vi "Cmd HO (TT).vi"(8 "error in (no error)":errorcluster caption="에러 입력(에러 없음)", 11 "AUDIX EM1000 입력":refnum<class "AUDIX EM1000.lvclass">) -> (0 "error out":errorcluster caption="에러 출력", 3 "AUDIX EM1000 출력":refnum<class "AUDIX EM1000.lvclass">)   [LabVIEW 2023, in "Turn Table and Mast.lvlib" / "AUDIX EM1000.lvclass"]
uses:
  AUDIX EM1000.lvclass
  AUDIX EM1000.lvclass/AUDIX EM1000.ctl
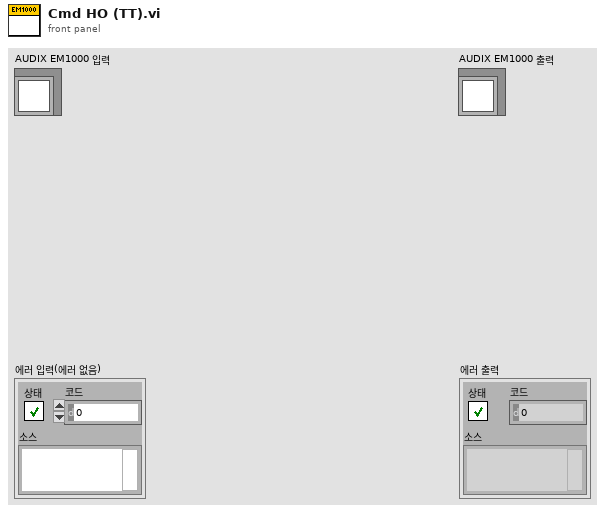
[diagram p1: front panel]
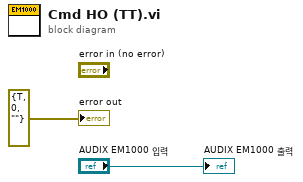
[diagram p0: block diagram]
diagram:
  "error out" <- errorcluster {"status"=TRUE, "code"=0, "source"=""} ("error out")
  "AUDIX EM1000 출력" <- "AUDIX EM1000 입력"
